vi "KYFG Set Camera Value Float.vi"(8 "error in (no error)":errorcluster, 9 "value":dbl, 10 "paramName":string, 11 "camHandle":u32) -> (0 "error out":errorcluster, 3 "camHandle out":u32)   [LabVIEW 2023, in "KYFGLib_lv.lvlib"]
doc: "KYFG_API FGSTATUS KYFG_SetCameraValue(CAMHANDLE camHandle, const char *paramName, void *paramValue);"
uses:
  KYFGLib_lv.lvlib
  KYFGLib.dll
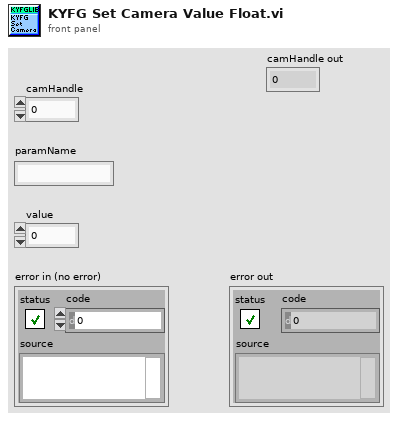
[diagram p1: front panel]
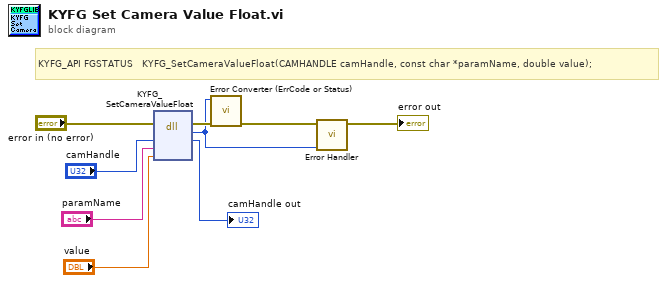
[diagram p0: block diagram]
diagram:
  # "KYFG_API FGSTATUS   KYFG_SetCameraValueFloat(CAMHANDLE camHandle, const char *paramName, double value);"
  n1 = dll-call lib="KYFGLib.dll" fn="KYFG_SetCameraValueFloat"(error in="error in (no error)", "camHandle"="camHandle", "paramName"="paramName", "paramValue"="value") -> (error out=w5:errorcluster, "return type"=w4:u32, "camHandle"=→"camHandle out":u32)  [unwired: 4 in, 1 out]
  n2 = call "Error Converter (ErrCode or Status).vi"("error in (no error)"=w5, "error code"=w4) -> ("error out"=w3:errorcluster)  [unwired: 9 in]
  n3 = call "Error Handler.vi"("Return Code"=w4, "Error In"=w3) -> ("Error Out"=→"error out":errorcluster)  [unwired: 9 in]
